vi "Initialize.vi"(8 "error in (no error)":errorcluster, 11 "Node name":string) -> (0 "error out":errorcluster)   [LabVIEW 2021, in "Iceoryx.lvlib"]
uses:
  Iceoryx.lvlib
  <vilib>/CIF Foundation/CIF Utilities/File/SubVIs/File Not Found Error Core.vi
  SubVIs/Convert Error Core.vi
  <vilib>/CIF Foundation/CIF Utilities/File/File_CIF_U.lvlib
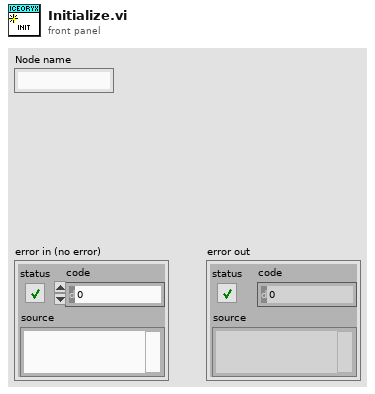
[diagram p1: front panel]
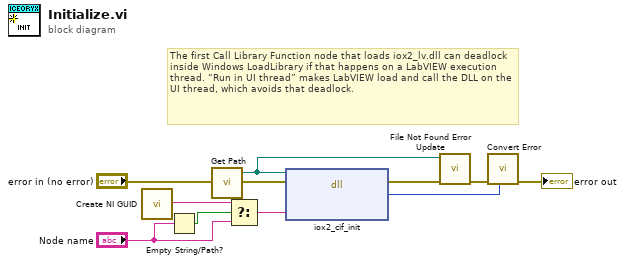
[diagram p0: block diagram]
diagram:
  # "The first Call Library Function node that loads iox2_lv.dll can deadlock inside Windows LoadLibrary if that happens on a LabVIEW execution thread. “Run in UI thread” makes LabVIEW load and call the DLL on the UI thread, which avoids that deadlock."
  n1 = call <vilib>:"Create NI GUID.vi"() -> ("NI GUID"=w3:string)
  n2 = Empty String/Path?(string/path="Node name") -> (empty?=w4:bool)
  n3 = call "Get Path.vi"() -> ("libiox2_cif path"=w5:path)  [unwired: 4 in]
  n4 = Select(t=w3, s=w4, f="Node name") -> (s? t:f=w2:string)
  n5 = dll-call lib="D:/dev/iceoryx2_lvwrapper/dist/iox2_cif.dll" fn="iox2_cif_init"(path in=w5, error in="error in (no error)", "node_name"=w2) -> (error out=w9:errorcluster, "return type"=w6:i32)  [unwired: 2 in, 1 out]
  n6 = call <vilib>:"File Not Found Error Update.vi"("error in"=w9, "path in"=w5) -> ("error out"=w8:errorcluster)  [unwired: 9 in]
  n7 = call "Convert Error.vi"("return type"=w6, "error in (no error)"=w8) -> ("error out"=→"error out":errorcluster)  [unwired: 9 in]
